vi "UE_Sweep_Target.vi"(3 "point_index":dbl, 4 "step_size":dbl, 5 "start_value":dbl) -> (2 "target":dbl)   [LabVIEW 2026]
doc: "INTENT: Compute start plus index times increment for a validated linear sweep. INPUTS: start_value (double), step_size (double), point_index (double). OUTPUTS: target (double). DESIGN CONSTRAINT: Sequencer validates point index and sweep size. REQUIREMENTS: SRS-F-019. No physical hardware side effects. Acceptance requires native LabVIEW compilation and behavioral testing."
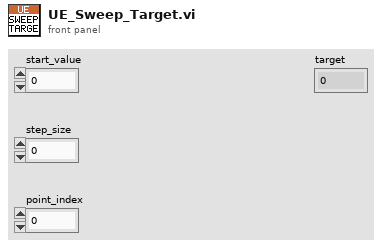
[diagram p1: front panel]
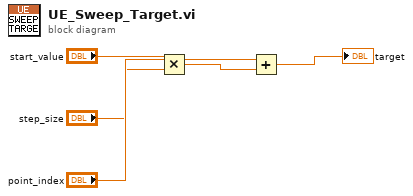
[diagram p0: block diagram]
diagram:
  n1 = Multiply(x="point_index", y="step_size") -> (x*y=w4:dbl)
  n2 = Add(x="start_value", y=w4) -> (x+y=→"target":dbl)
